vi "GpuMat CreateRoi.vi"(8 "error in (no error)":errorcluster, 9 "Size":T1, 10 "TopLeft":T1, 11 "GpuMat":refnum<class "GpuMat.lvclass">) -> (0 "error out":errorcluster, 2 "Header out":refnum<class "GpuMat.lvclass">, 3 "GpuMat out":refnum<class "GpuMat.lvclass">)   [LabVIEW 2020, in "OpenLvVision_OpenCv.lvlib" / "Cuda.lvlib" / "GpuMat.lvclass"]
doc: "Object by reference!\n\nCreates a GpuMat header for a part of the bigger matrix"
uses:
  GpuMat.lvclass
  C:/Users/lukas/Documents/OpenLvVision_OpenCv/SourceCode/LabView/OpenLvVision_OpenCv/_LvHelpers/EdvrObject/EdvrObject.lvclass
  TypeDef/Point/2D_PointI32.ctl
  _LvHelpers/EdvrObject/EdvrObject.lvclass/EdvrObject.ctl
  _LvHelpers/EdvrObject/TypeDef/Edvr.ctl
  _LvHelpers/EdvrObject/EdvrObject.lvclass
  OpenLvVision_OpenCv.lvlib
  <vilib>/Utility/error.llb/Error Cluster From Error Code.vi
  <vilib>/ErrorRing/Error Ring.xnode
  Dlls/OlvOpenCvWrapper.dll
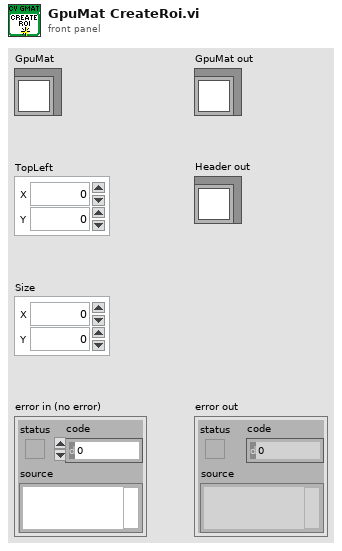
[diagram p1: front panel]
types:
  T1 = typedef "OpenLvVision_OpenCv.lvlib/2D_PointI32.ctl" = cluster{"X":i32, "Y":i32}
  T2 = typedef "OpenLvVision_OpenCv.lvlib/EdvrObject.lvclass/Edvr.ctl" = refnum<data-value>
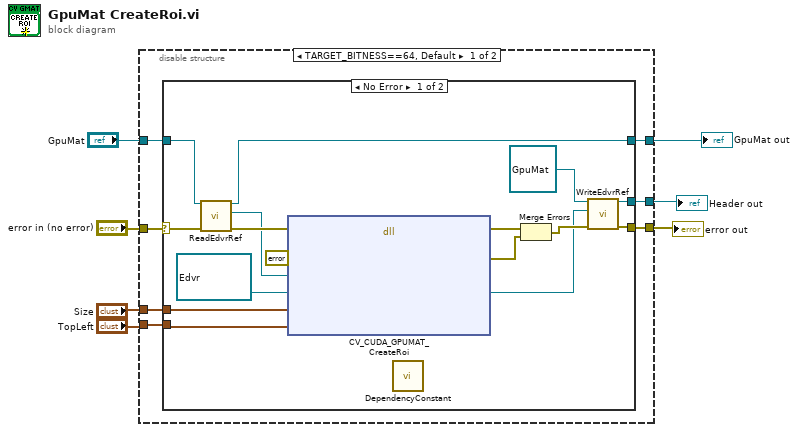
[diagram p0: block diagram]
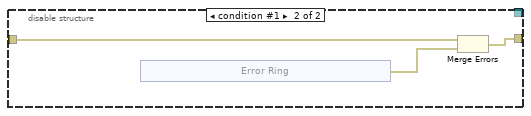
[diagram p3: hidden frame]
diagram:
  n1 = disable-structure shown="TARGET_BITNESS==64, Default" {
    disable-tunnel: "error in (no error)" -> [w14 w34]
    disable-tunnel: [w13 _] -> w5
    disable-tunnel: [w12 w35] -> w7
    disable-tunnel: "GpuMat" -> [w11 _]
    disable-tunnel: [w10 _] -> w3
    disable-tunnel: "TopLeft" -> [w9 _]
    disable-tunnel: "Size" -> [w8 _]
    frame condition #0 (active) {
      n2 = case shown="No Error" w14 {
        selector: w14 -> [w21 w32]
        tunnel: [w30 w32] -> w12
        tunnel: [w29 _] -> w13
        tunnel: w11 -> [w19 w31]
        tunnel: [w17 w31] -> w10
        tunnel: w9 -> [w15 _]
        tunnel: w8 -> [w16 _]
        frame No Error {
          n3 = call "ReadEdvrRef.vi"("error in (no error)"=w21, "EdvrObject in"=w19) -> ("error out"=w20:errorcluster, "Edvr"=w18:T2, "EdvrObject out"=w17:refnum<class "GpuMat.lvclass">)  [unwired: 7 in]
          n4 = dll-call lib="C:/Users/lukas/Documents/OpenLvVision_OpenCv/SourceCode/LabView/OpenLvVision_OpenCv/Dlls/OlvOpenCvWrapper.dll" fn="CV_CUDA_GPUMAT_CreateRoi"(error in=w20, "Error"=errorcluster {"status"=FALSE, "code"=0, "source"=""} ("error out"), "srcRef"=w18, "dstRef"=T2 refnum ("Edvr"), "Size"=w16, "topLeft"=w15) -> (error out=w27:errorcluster, "Error"=w26:errorcluster, "dstRef"=w23:T2)  [unwired: 6 in, 1 out]
          n5 = call "DependencyConstant.vi"() -> ()  [unwired: 12 in]
          n6 = Merge Errors(w27, w26) -> (w24:errorcluster)
          n7 = call "WriteEdvrRef.vi"("error in (no error)"=w24, "Edvr"=w23, "EdvrObject in"=refnum<class "GpuMat.lvclass"> refnum ("OpenLvVision_OpenCv.lvlib:Cuda:GpuMat")) -> ("error out"=w30:errorcluster, "EdvrObject out"=w29:refnum<class "GpuMat.lvclass">)  [unwired: 7 in]
        }
        frame Error {
        }
      }
    }
    frame condition #1 {
      n8 = xnode "Error Ring"() -> ("error out"=w33:errorcluster)
      n9 = Merge Errors(w34, w33) -> (w35:errorcluster)
    }
  }
  "error out" <- w7
  "GpuMat out" <- w3
  "Header out" <- w5
